vi "Read INI Table.vi"(8 "error in (no error)":errorcluster, 10 "Keys":string[](array[string]), 11 "File Path":path) -> (0 "error out":errorcluster, 2 "Values":string[][](array[string]), 3 "Section Names":string[](array[string]))   [LabVIEW 2024]
doc: "Reads a schema-version-2 INI file as a table. Every section except [_Meta] is a row; Section Names returns the row keys (GUIDs) in file order and Values returns one row per section holding the value of each of the given Keys as text (strings without their quotes, booleans as TRUE/FALSE, numbers as written). A key that is missing reads as an empty string. A file that does not exist gives two empty arrays and no error.\n\nGenerated by: Claude"
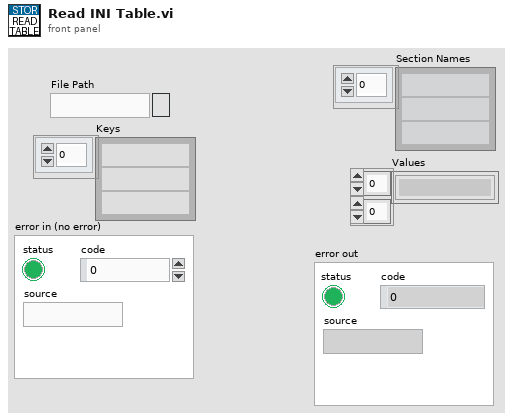
[diagram p1: front panel]
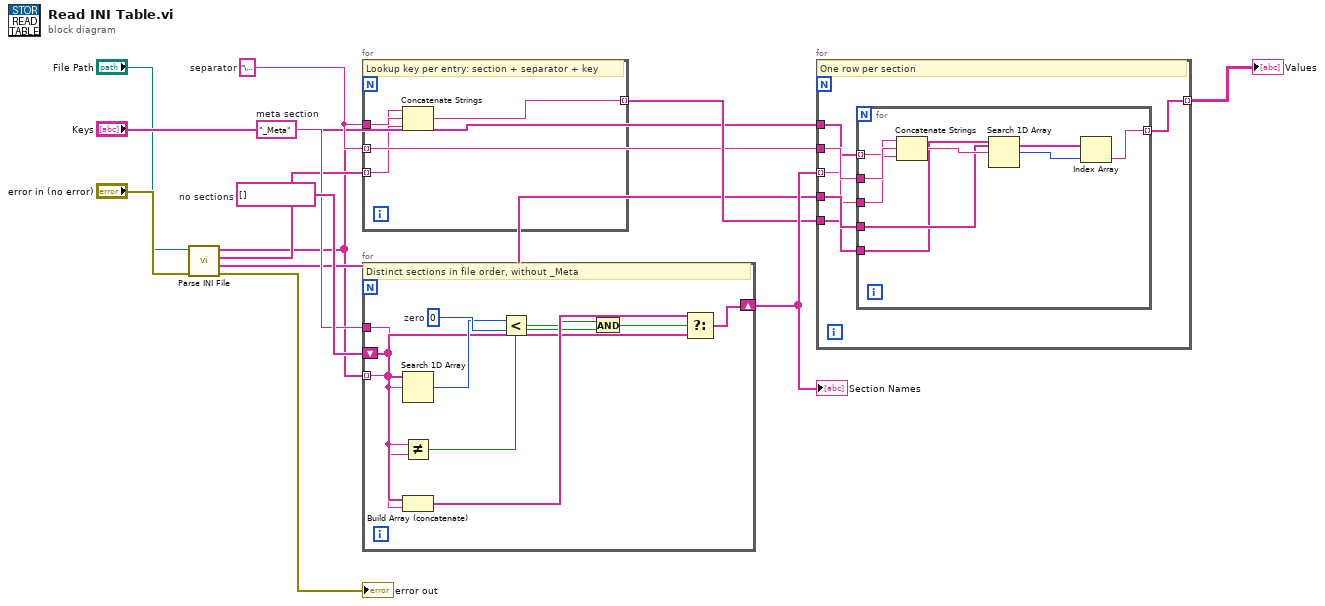
[diagram p0: block diagram]
diagram:
  w10 = string[] []  # no sections
  w9 = "_Meta"  # meta section
  w8 = "\u0001"  # separator
  n1 = call "Parse INI File.vi"("error in (no error)"="error in (no error)", "File Path"="File Path") -> ("error out"=→"error out":errorcluster, "Values"=w6:string[], "Keys"=w5:string[], "Sections"=w4:string[])  [unwired: 6 in]
  n2 = for {
    tunnel: w8 -> [w16]
    tunnel: w4 -> [w14] mode=indexing
    tunnel: w5 -> [w15] mode=indexing
    tunnel: [w17] -> w11 mode=indexing
    # "Lookup key per entry: section + separator + key"
    n3 = Concatenate Strings(w14, w16, w15) -> (w17:string)
  }
  n4 = for {
    tunnel: w9 -> [w19]
    shift-right: [w21] -> w12
    shift-left: w10 -> [w20]
    tunnel: w4 -> [w18] mode=indexing
    w23 = 0  # zero
    # "Distinct sections in file order, without _Meta"
    n5 = Search 1D Array(1D array=w20, element=w18) -> (index of element=w22:i32)  [unwired: 1 in]
    n6 = Not Equal?(x=w18, y=w19) -> (x != y?=w25:bool)
    n7 = Build Array (concatenate)(w20, w18) -> (w27:string[])
    n8 = Less?(x=w22, y=w23) -> (x < y?=w24:bool)
    n9 = And(x=w24, y=w25) -> (x .and. y?=w26:bool)
    n10 = Select(t=w27, s=w26, f=w20) -> (s? t:f=w21:string[])
  }
  "Section Names" <- w12
  n11 = for {
    tunnel: "Keys" -> [w29]
    tunnel: w8 -> [w32]
    tunnel: w12 -> [w28] mode=indexing
    tunnel: w6 -> [w31]
    tunnel: w11 -> [w30]
    tunnel: [w33] -> w13 mode=indexing
    # "One row per section"
    n12 = for {
      tunnel: w29 -> [w34] mode=indexing
      tunnel: w32 -> [w38]
      tunnel: w28 -> [w35]
      tunnel: w31 -> [w37]
      tunnel: w30 -> [w36]
      tunnel: [w41] -> w33 mode=indexing
      n13 = Concatenate Strings(w35, w38, w34) -> (w39:string)
      n14 = Search 1D Array(1D array=w36, element=w39) -> (index of element=w40:i32)  [unwired: 1 in]
      n15 = Index Array(array=w37, index=w40) -> (element=w41:string)
    }
  }
  "Values" <- w13
